vi "RemoteVI Wait Input Handled.vi"(0 "hWnd":u64, 11 "error in":errorcluster) -> (15 "error out":errorcluster)   [LabVIEW 2020, in "RemoteVI.lvlib"]
doc: "Waits until the thread of hWnd (LabVIEW's UI thread) has handled the messages posted to it so far, at most about 1 s. LabVIEW drops and reorders key messages that arrive in a burst - twelve posted Backspace key-downs became one, and the generated WM_CHAR of a key-down landed behind characters posted after it (measured) - and decides how to read a button-up from the mouse capture its button-down set up (RemoteVI Mouse Captured.vi). So RemoteVI Post Input.vi posts each message only after LabVIEW has finished the one before. Mechanism: a SENT message is delivered when the receiving thread next looks into its queue, before any posted message is returned, so the first WM_NULL sent with user32 SendMessageTimeoutW.vi returns once LabVIEW has fetched the queued posts, and the second once it has come back for more - after handling them. SMTO_ABORTIFHUNG, 500 ms each; a timeout (a busy or hung UI thread) is not an error, the caller just goes on. Sent messages are also handled inside LabVIEW's modal loops (popup menus, mouse tracking), so this never deadlocks. An incoming error skips the work."
uses:
  RemoteVI.lvlib
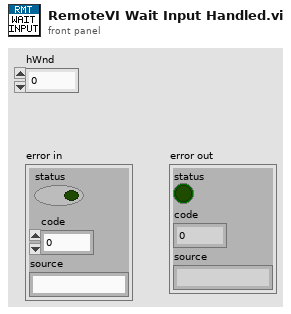
[diagram p1: front panel]
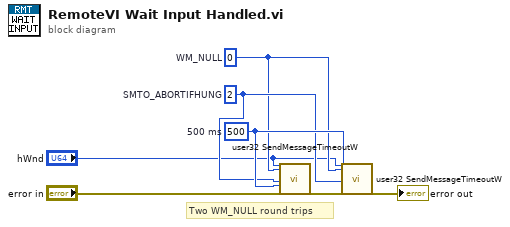
[diagram p0: block diagram]
diagram:
  w5 = u32 500  # 500 ms
  w4 = u32 2  # SMTO_ABORTIFHUNG
  w3 = u32 0  # WM_NULL
  # "Two WM_NULL round trips"
  n1 = call "user32 SendMessageTimeoutW.vi"("hWnd"="hWnd", "Msg"=w3, "fuFlags"=w4, "uTimeout"=w5, "error in"="error in") -> ("error out"=w6:errorcluster)  [unwired: 20 in, 2 out]
  n2 = call "user32 SendMessageTimeoutW.vi"("hWnd"="hWnd", "Msg"=w3, "fuFlags"=w4, "uTimeout"=w5, "error in"=w6) -> ("error out"=→"error out":errorcluster)  [unwired: 20 in, 2 out]
